vi "VIH ProjFile - Path Converter - Read.vi"(11 "Path in":path) -> (3 "Path out":path)   [LabVIEW 2014]
doc: "::: VI Helpeks :::\nCopyright (c) 2000-2026 Konstantin Shifershteyn. All rights reserved."
panel:
  # "VI Helpeks\nCopyright (c) 2012-2026 Konstantin Shifershteyn"
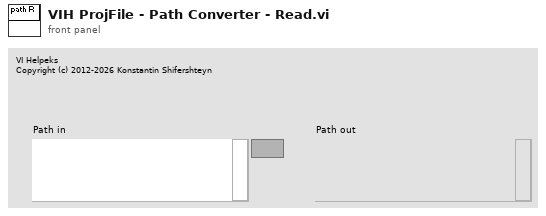
[diagram p1: front panel]
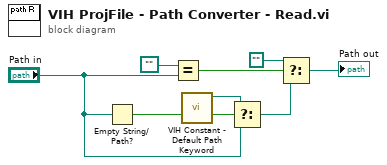
[diagram p0: block diagram]
diagram:
  n1 = Empty String/Path?(string/path="Path in") -> (empty?=w6:bool)
  n2 = Equal?(x=path "" ("y"), y="Path in") -> (x = y?=w8:bool)
  n3 = call "VIH Constant - Default Path Keyword.vi"() -> ("<default> path"=w1:path)  [unwired: 11 in]
  n4 = Select(t=w1, s=w6, f="Path in") -> (s? t:f=w5:path)
  n5 = Select(t=path "", s=w8, f=w5) -> (s? t:f=→"Path out":path)
